vi "Acquisition.vi"(7 "CSM Name":string="CSM-Module") -> ()   [LabVIEW 2026, in "UI-压力.lvlib" / "Acquisition.lvlib"]
uses:
  Acquisition.lvlib
  Supports/Acquiring States.ctl
  Supports/Device Info.ctl
  Data ColndSave/Supports/Time and Data.ctl
  7c1bd55a-2ec8-456f-bad7-7e130b55c93f.vi
  d2ac0b8d-a34d-4c44-96e2-60a2cc9ef1dc.vi
  144ef8d5-f062-4612-a884-90947adc4c96.vi
  <userlib>/_NEVSTOP/Communicable State Machine(CSM)/AdvanceAPI/CSM - Revert Arguments-Safe String.vi
  <userlib>/_NEVSTOP/Communicable State Machine(CSM)/_Shared/Trim Single-line Text.vi
  <userlib>/_NEVSTOP/Communicable State Machine(CSM)/AdvanceAPI/CSM - Make String Arguments Safe.vi
  <userlib>/_NEVSTOP/Communicable State Machine(CSM)/AdvanceAPI/CSM - Break Down Multiple States String.vi
  <userlib>/_NEVSTOP/Communicable State Machine(CSM)/AdvanceAPI/CSM - Compact Multiple States.vi
  <userlib>/_NEVSTOP/Communicable State Machine(CSM)/AdvanceAPI/CSM - Keywords.vi
  <userlib>/_NEVSTOP/Communicable State Machine(CSM)/addons/API-String-Arugments-Support/_Support/Convert API String Arguments to Data(variant).vi
  <vilib>/Instr/_visa.llb/VISA Configure Serial Port (Instr).vi
  <userlib>/_NEVSTOP/Communicable State Machine(CSM)/addons/MassData-Parameter/_support/FGV-MassData(lvlibp).vi
  <userlib>/_NEVSTOP/Communicable State Machine(CSM)/Communicable State Machine.lvlib
  <userlib>/_NEVSTOP/Communicable State Machine(CSM)/addons/Loop-Support/CSM Loop Support.lvlib
  Data ColndSave/Data Collection and Save.lvlib
panel:
  out "Error Occurred":errorcluster
  out "State History":string
  in  "Exit":bool
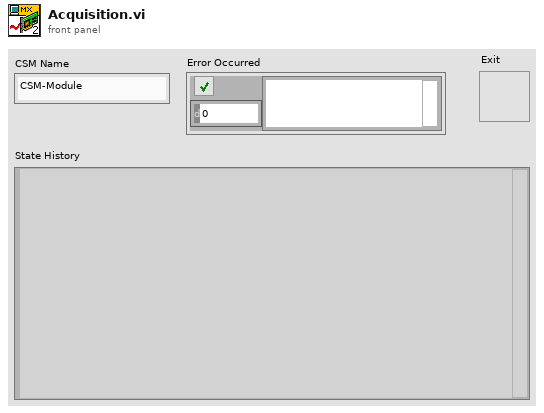
[diagram p1: front panel]
types:
  T1 = enum32{"Invalid", "Standard", "Closed", "Hidden", "Minimized", "Maximized"}
  T2 = enum32{"invalid app kind", "Development System", "Run Time System", "Student Edition", "Embedded LabVIEW", "Evaluation", "Custom"}
  T3 = typedef "UI-压力.lvlib/Acquisition.lvlib/Acquiring States.ctl" = enum16{"Idle", "Acquiring", "Error"}
  T4 = cluster{"波特率":u32, "数据位":u16, "校验":enum16{"None", "Odd", "Even", "Mark", "Space"}, "停止位":u16, "流控制":u16}
  T5 = typedef "Communicable State Machine.lvlib/_CSM_Response Source Message.ctl" = cluster{"‘State":string, "’Arguments":string, "’Error":errorcluster}
  T6 = cluster{"Current VI Reference":refnum<vi>, "Close Panel on Exit?":bool}
  T7 = typedef "UI-压力.lvlib/Device Info.ctl" = cluster{"USB Port":refnum<visa-resource-name>, "采集间隔(s)":dbl, "压力设备选择":bool}
  T8 = cluster{"Core":cluster{"Current VI Reference":refnum<vi>, "Close Panel on Exit?":bool}, "State":T3, "基本信息":T7, "采集时间":timestamp}
  T9 = typedef "Data Collection and Save.lvlib/Time and Data.ctl" = cluster{"采集时间":timestamp, "Data":dbl[]}
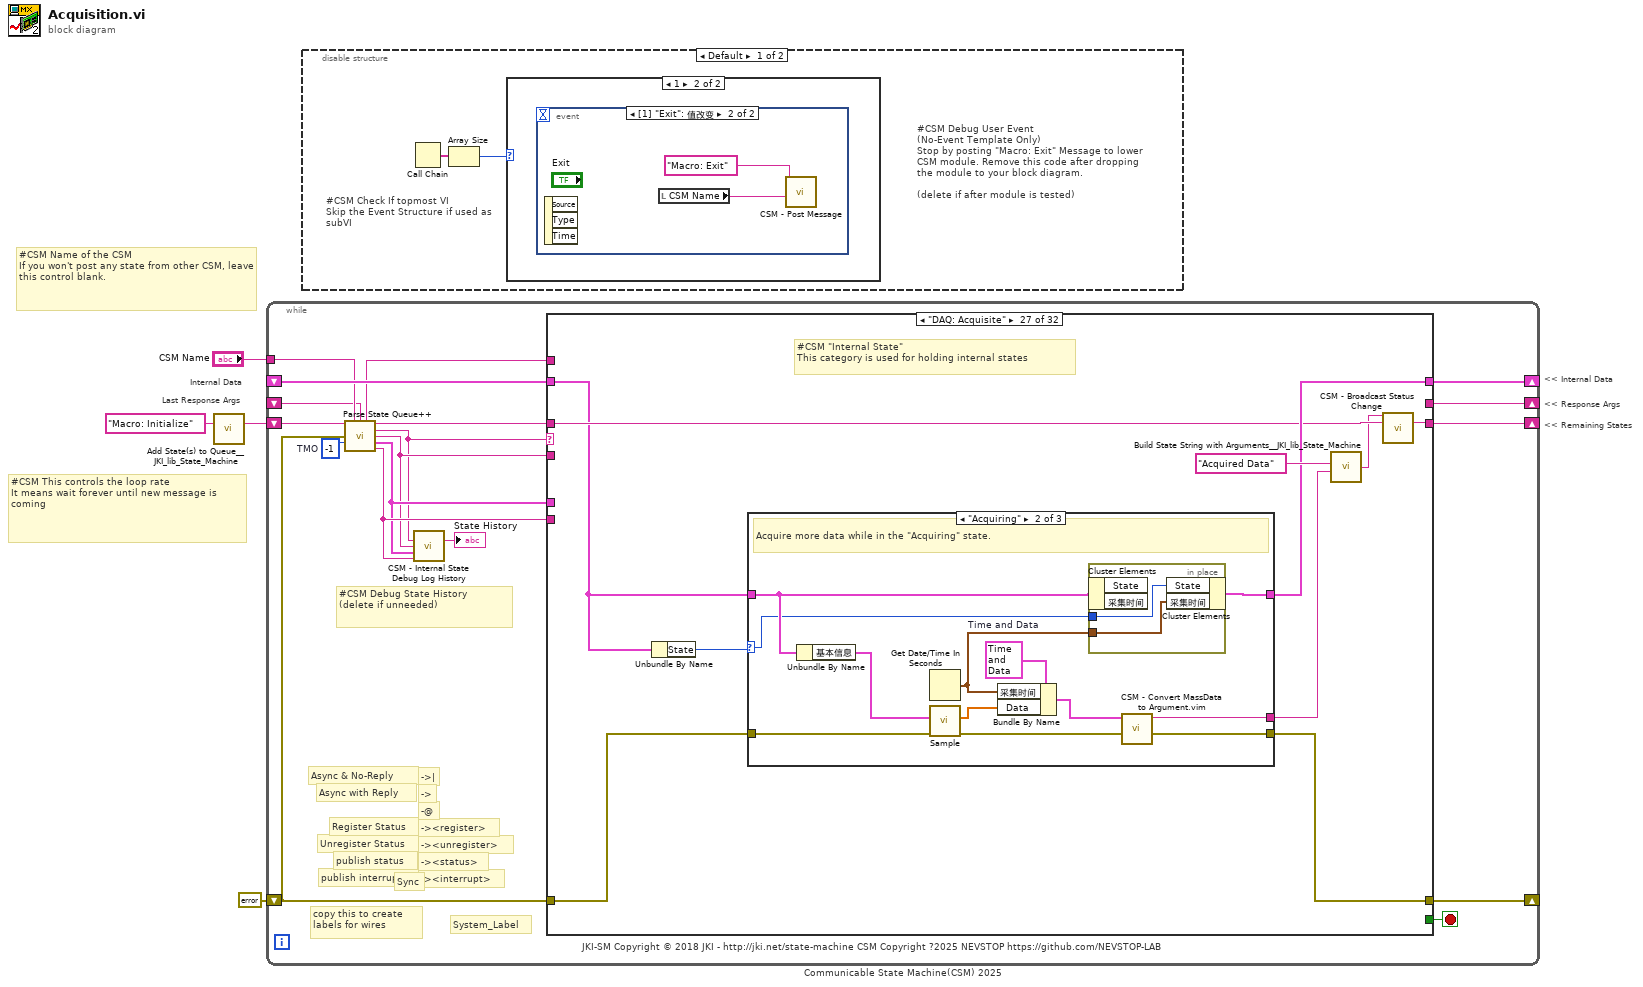
[diagram p0: block diagram]
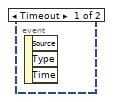
[diagram p3: hidden frame]
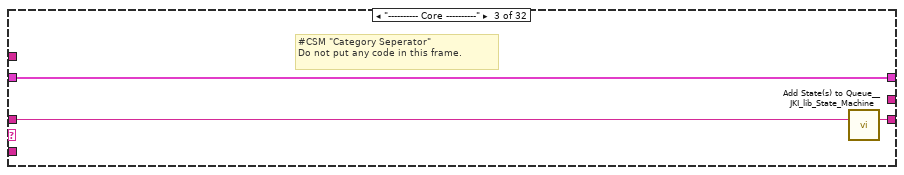
[diagram p7: hidden frame]
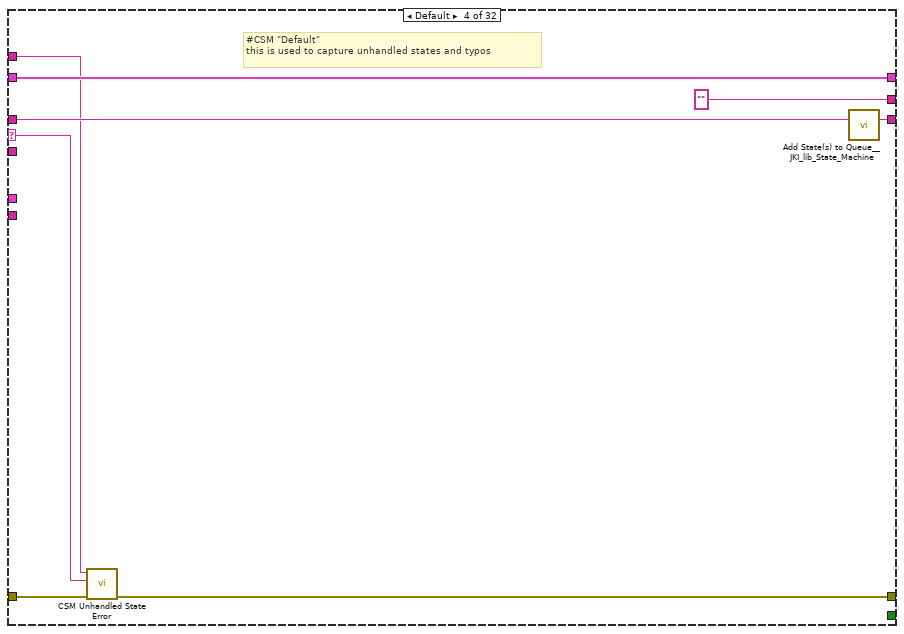
[diagram p8: hidden frame]
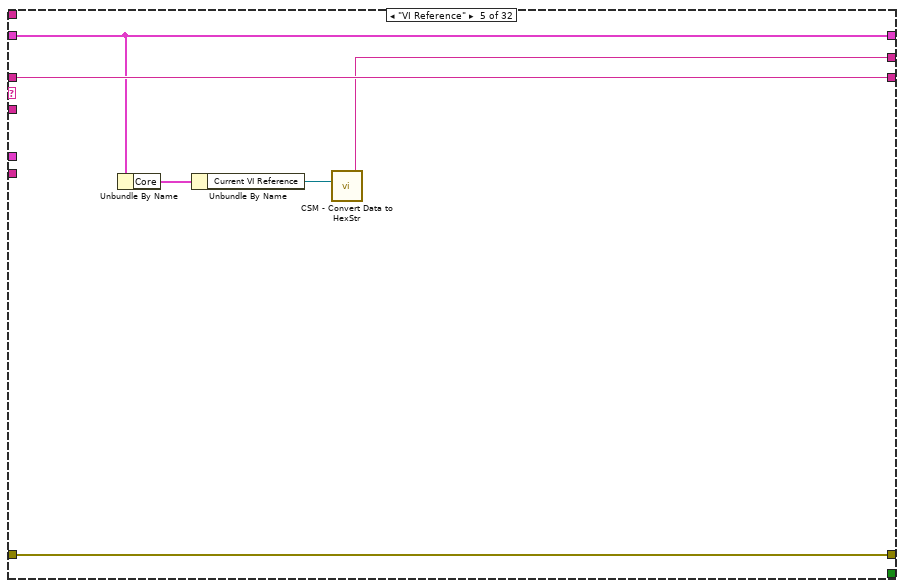
[diagram p9: hidden frame]
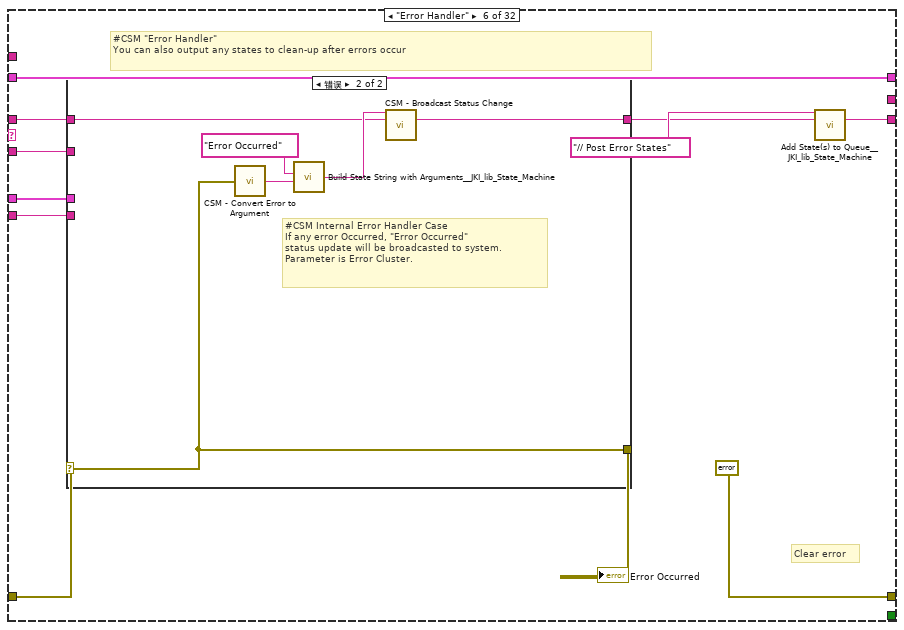
[diagram p10: hidden frame]
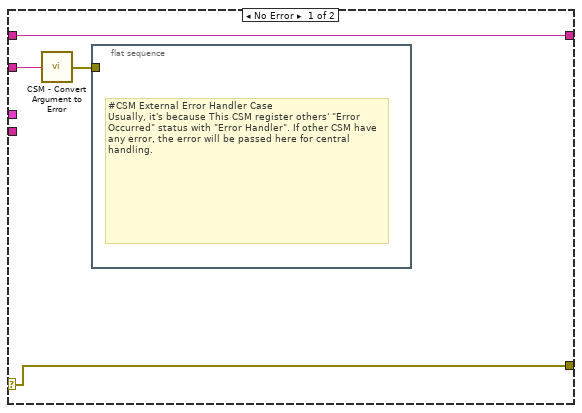
[diagram p11: hidden frame]
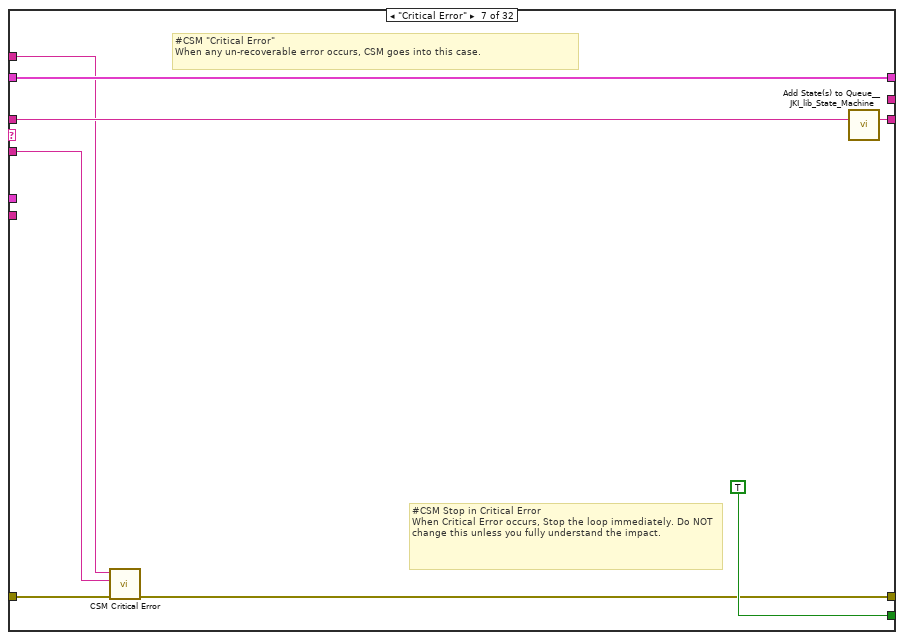
[diagram p12: hidden frame]
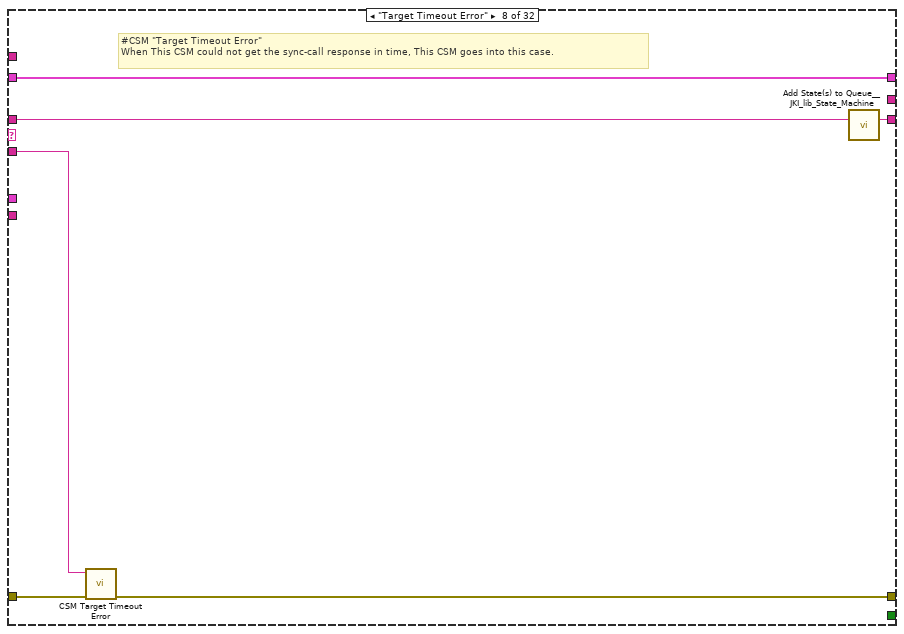
[diagram p13: hidden frame]
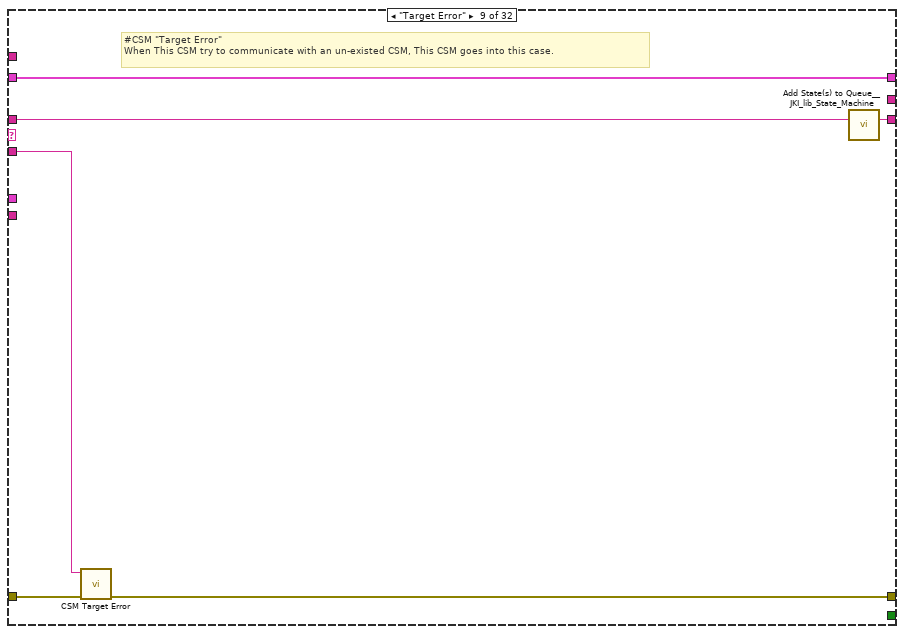
[diagram p14: hidden frame]
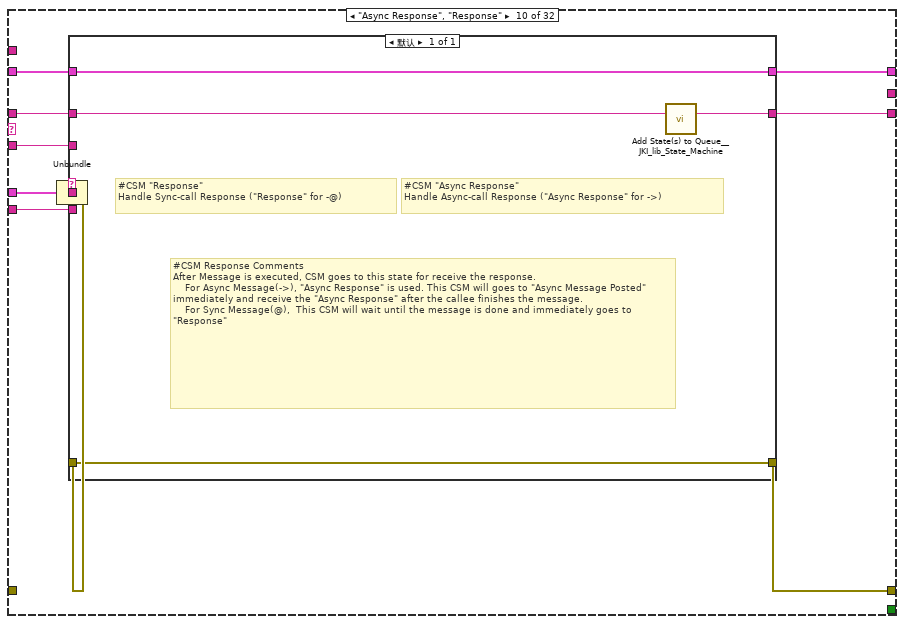
[diagram p15: hidden frame]
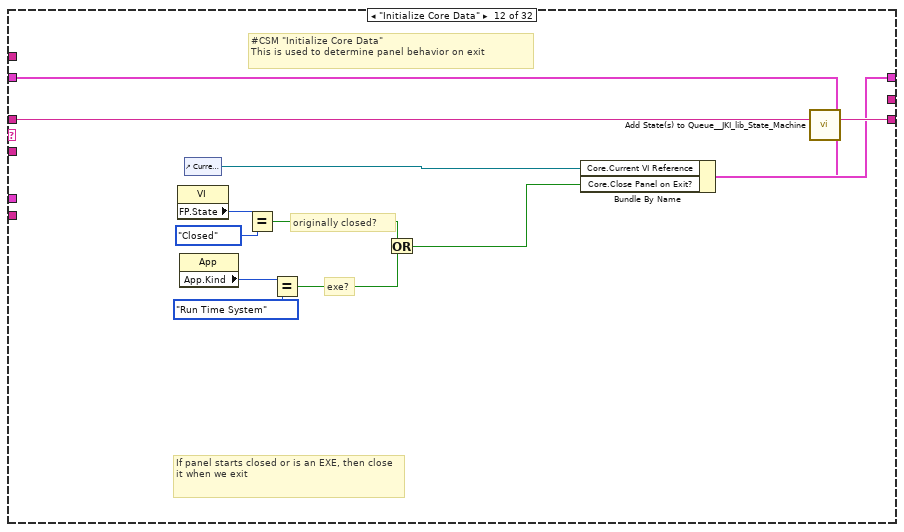
[diagram p17: hidden frame]
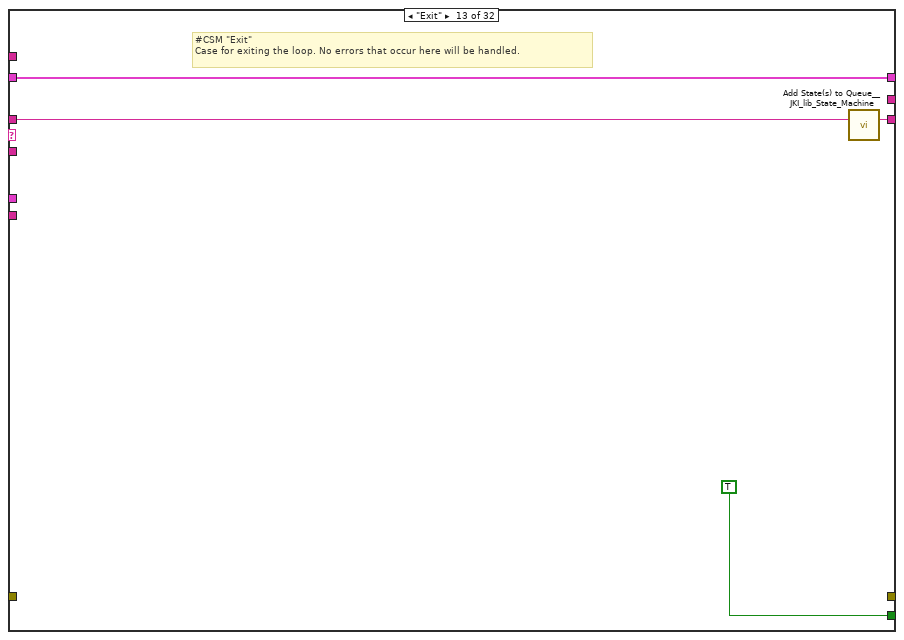
[diagram p18: hidden frame]
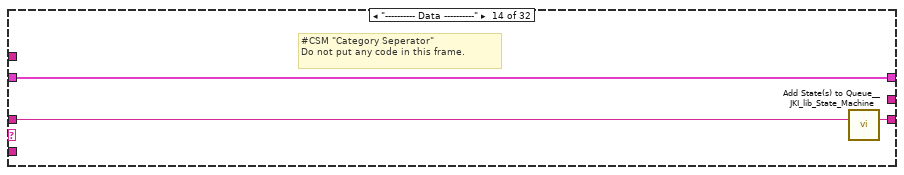
[diagram p19: hidden frame]
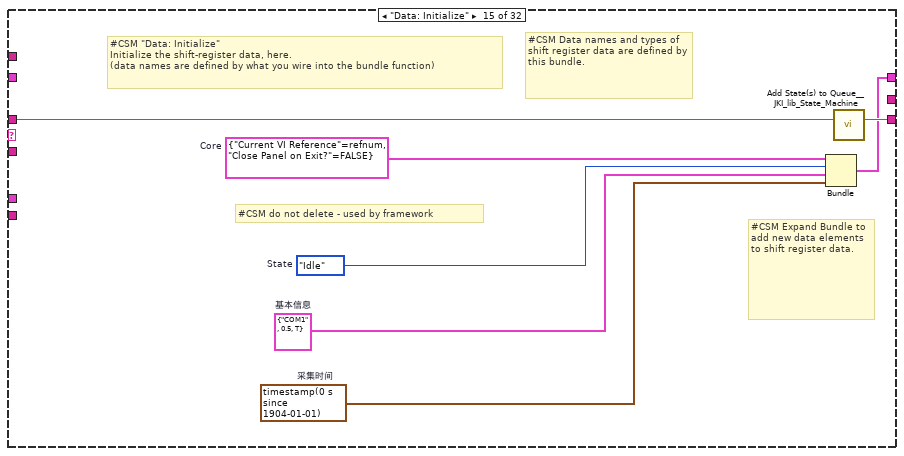
[diagram p20: hidden frame]
diagram:
  # "Last Response Args"
  # "Internal Data"
  # "#CSM Name of the CSM\nIf you won't post any state from other CSM, leave this control blank."
  # "#CSM This controls the loop rate\nIt means wait forever until new message is coming"
  # "<< Internal Data"
  # "<< Response Args"
  # "<< Remaining States"
  n1 = call <vilib>:"Add State(s) to Queue__JKI_lib_State_Machine.vi"("State(s) in (\"\")"="Macro: Initialize" ("Init State(\"Macro: Initialize\")")) -> ("States Out"=w1:string)  [unwired: 14 in]
  n2 = while "Communicable State Machine(CSM) 2025" {
    shift-right: [w17] -> _
    shift-left: _ -> [w16]
    shift-right: [w20] -> _
    shift-left: errorcluster {"status"=FALSE, "code"=0, "source"=""} ("error out") -> [w6]
    shift-right: [w19] -> _
    shift-left: w1 -> [w21]
    tunnel: "CSM Name" -> [w13]
    shift-right: [w14] -> _
    shift-left: _ -> [w8]
    stop <- w18 stop-if-true
    w15 = -1  # TMO
    # "#CSM Debug State History\n(delete if unneeded)"
    # "-><interrupt>"
    # "-><status>"
    # "-><unregister>"
    # "-><register>"
    # "-@"
    # "->"
    # "->|"
    # "publish interrupt"
    # "publish status"
    # "Unregister Status"
    # "Register Status"
    # "Sync"
    # "Async with Reply"
    # "Async & No-Reply"
    # "JKI-SM Copyright © 2018 JKI - http://jki.net/state-machine CSM Copyright ?2025 NEVSTOP https://github.com/NEVSTOP-LAB"
    # "copy this to create labels for wires"
    # "System_Label"
    n3 = call <userlib>:"Parse State Queue++.vi"("State Queue"=w21, "Name (\"\" to Use UUID)"=w13, "Response Arguments"=w8, "Previous Error"=w6, "Dequeue (1 ms)"=w15) -> ("Name Used"=w7:string, "Remaining States"=w22:string, "Current State"=w9:string, "Arguments"=w10:string, "Additional Information"=w11:T5, "Source CSM"=w12:string)  [unwired: 5 in]
    n4 = call <userlib>:"CSM - Internal State Debug Log History.vi"("State"=w9, "Arguments (\"\")"=w10, ">> Response Source Message >>"=w11, "Source (\"\")"=w12) -> ("Debug Log"=→"State History":string)  [unwired: 11 in]
    n5 = case shown="\"DAQ: Acquisite\"" w9 {
      selector: w9 -> [_ _ _ w33 _ _ _ _ _ _ _ _ _ _ _ _ _ _ _ _ _ _ _ _ _ _ _ _ _ _ w269 _]
      tunnel: w22 -> [w23 w26 w29 w37 w42 w48 w72 w78 w84 w94 w101 w113 w117 w120 w127 w130 w136 w139 w144 w153 w158 w163 w177 w182 w192 w205 w216 w247 w256 w258 w271 w274]
      tunnel: w10 -> [_ _ _ _ _ w47 w68 w75 w81 w88 _ _ _ _ _ _ _ _ _ _ _ w160 _ w186 _ _ _ _ _ _ w268 _]
      tunnel: w16 -> [w24 w25 w27 w35 w41 w53 w70 w76 w82 w92 w100 w107 w115 w118 _ w129 w131 w137 w142 w147 w157 w164 w179 w185 w190 w203 w213 w242 w253 w257 w260 w275]
      tunnel: [_ _ _ w30 w43 errorcluster {"status"=FALSE, "code"=0, "source"=""} ("error out") w65 w73 w79 w95 _ _ _ _ _ _ w132 _ w140 w145 _ w159 w175 w189 _ _ w218 _ _ w259 w272 w276] -> w20
      tunnel: w6 -> [_ _ _ w31 w43 w51 w66 w74 w80 _ _ _ _ _ _ _ w133 _ w140 w145 _ w159 w175 w189 _ _ w217 w241 _ w259 w272 w276]
      tunnel: [w23 w26 w28 w36 w42 w49 w71 w77 w83 w93 w101 w112 w116 w119 w126 w130 w135 w138 w143 w152 w158 w162 w178 w183 w191 w204 w214 w246 w255 w258 w270 w273] -> w19
      tunnel: [_ _ _ _ _ _ TRUE _ _ _ _ _ TRUE _ _ _ _ _ _ _ _ _ _ _ _ _ _ _ _ _ _ _] -> w18
      tunnel: [w24 w25 w27 w35 w41 w53 w70 w76 w82 w91 w100 w111 w115 w118 w125 w129 w131 w137 w142 w147 w157 w161 w179 w184 w190 w202 w219 w242 w252 w257 w260 w275] -> w17
      tunnel: w12 -> [_ _ _ _ _ w46 _ _ _ w89 _ _ _ _ _ _ _ _ _ _ _ _ _ _ _ _ _ _ _ _ _ _]
      tunnel: w11 -> [_ _ _ _ _ w45 _ _ _ w90 _ _ _ _ _ _ _ _ _ _ _ _ _ _ _ _ _ _ _ _ _ _]
      tunnel: [_ _ _ "" w38 _ _ _ _ _ _ _ _ _ _ _ _ _ _ _ _ _ _ _ _ _ _ _ _ _ _ _] -> w14
      tunnel: w7 -> [_ _ _ w32 _ _ w67 _ _ _ _ _ _ _ _ _ _ _ _ _ _ _ _ _ _ _ _ _ _ _ _ _]
      frame "", "Idle" {
        # "#CSM \"Idle/Event Handler\"\nexecutes when the state queue is empty"
      }
      frame "CSM Documentation" {
        # "#CSM State Syntax\n\n// Comment line, all text to the right of “//” will be ignored\n// Local Message Example\nDoSth: DoA >> Arguments\n\n// Sync Call Example\nAPI: xxxx >> Arguments -@ TargetModule\n\n// Async Call Example\nAPI: xxxx >> Arguments -> TargetModule\n\n// Async Call without Reply Example\nAPI: xxxx >> Arguments ->| TargetModule\n\n// Broadcast normal status:\nStatus >> StatusArguments  -><status>\n\n// Broadcast Interrupt status:\nInterrupt >> StatusArguments  -><interrupt>\n\n// Register Source Module's status to Handler Module\nStatus@Source Module >> Handler Module@Handler Module -><register>\n\n// Unegister Source Module's status\nStatus@Source Module >> Handler Module -><unregister>"
        # "#CSM README FIRST\n\nCommunicable State Machine(CSM) is a LabVIEW application framework that builds upon JKI State Machine(JKISM). It follows the pattern of JKISM and extends the keywords to describe message communication between modules, including concepts such as Sync-Message, Async-Message, Subscription/Unsubscription of status - essential elements for creating reusable code modules. For more information, please visit the CSM wiki: https://nevstop-lab.github.io/CSM-Wiki/\n\nFor instructions on JKI State Machine, visit: \n    http://jki.net/state-machine/\nFor information about CSM, visit: \n    https://github.com/NEVSTOP-LAB"
        # "#CSM \"Documentation\"\nCase for holding CSM Documenation"
      }
      frame "---------- Core ----------" {
        # "#CSM \"Category Seperator\"\nDo not put any code in this frame."
        n6 = call <vilib>:"Add State(s) to Queue__JKI_lib_State_Machine.vi"("State(s) in (\"\")"=w29) -> ("States Out"=w28:string)  [unwired: 14 in]
      }
      frame Default {
        # "#CSM \"Default\"\nthis is used to capture unhandled states and typos"
        n7 = call <userlib>:"CSM Unhandled State Error.vi"("error in (no error)"=w31, "Undefined State"=w33, "CSM Name"=w32) -> ("error out"=w30:errorcluster)  [unwired: 8 in]
        n8 = call <vilib>:"Add State(s) to Queue__JKI_lib_State_Machine.vi"("State(s) in (\"\")"=w37) -> ("States Out"=w36:string)  [unwired: 14 in]
      }
      frame "VI Reference" {
        n9 = Unbundle By Name(w41) -> ("Core"=w40:T6)
        n10 = Unbundle By Name(w40) -> ("Current VI Reference"=w39:refnum<vi>)
        n11 = call <userlib>:"CSM - Convert Data to HexStr.vi"("Variant"=w39) -> ("HEX String (0-9,A-F)"=w38:string)  [unwired: 8 in]
      }
      frame "Error Handler" {
        # "#CSM \"Error Handler\"\nYou can also output any states to clean-up after errors occur"
        # "Clear error"
        n12 = case shown="错误" w51 {
          selector: w51 -> [w55 w59]
          tunnel: [w58 w61] -> w50
          tunnel: w48 -> [w58 w60]
          tunnel: w47 -> [w57 _]
          tunnel: w46 -> [_ _]
          tunnel: w45 -> [_ _]
          tunnel: [w55 w59] -> w44
          frame No Error {
            n13 = call <userlib>:"CSM - Convert Argument to Error.vi"("Argument"=w57) -> ("Error"=w56:errorcluster)  [unwired: 4 in]
            n14 = flat-sequence {
              tunnel: w56 -> [_]
              frame #0 {
                # "#CSM External Error Handler Case\nUsually, it's because This CSM register others' \"Error Occurred\" status with \"Error Handler\". If other CSM have any error, the error will be passed here for central handling."
              }
            }
          }
          frame Error {
            # "#CSM Internal Error Handler Case \nIf any error Occurred, \"Error Occurred\" \nstatus update will be broadcasted to system.\nParameter is Error Cluster."
            n15 = call <userlib>:"CSM - Convert Error to Argument.vi"("Error"=w59) -> ("Argument"=w63:string)  [unwired: 4 in]
            n16 = call <vilib>:"Build State String with Arguments__JKI_lib_State_Machine.vi"("Arguments (\"\")"=w63, "State"="Error Occurred" ("Status with Arguments")) -> ("State with Arguments"=w62:string)  [unwired: 4 in]
            n17 = call <userlib>:"CSM - Broadcast Status Change.vi"("Status With Arguments"=w62, "State Queue"=w60) -> ("Remaining States"=w61:string)  [unwired: 13 in]
          }
        }
        "Error Occurred" <- w44
        n18 = call <vilib>:"Add State(s) to Queue__JKI_lib_State_Machine.vi"("State(s) in Front (\"\")"="// Post Error States", "State(s) in (\"\")"=w50) -> ("States Out"=w49:string)  [unwired: 13 in]
      }
      frame "Critical Error" {
        # "#CSM \"Critical Error\"\nWhen any un-recoverable error occurs, CSM goes into this case."
        # "#CSM Stop in Critical Error\nWhen Critical Error occurs, Stop the loop immediately. Do NOT change this unless you fully understand the impact."
        n19 = call <userlib>:"CSM Critical Error.vi"("error in (no error)"=w66, "Arugments (As Reason)"=w68, "CSM Name"=w67) -> ("error out"=w65:errorcluster)  [unwired: 8 in]
        n20 = call <vilib>:"Add State(s) to Queue__JKI_lib_State_Machine.vi"("State(s) in (\"\")"=w72) -> ("States Out"=w71:string)  [unwired: 14 in]
      }
      frame "Target Timeout Error" {
        # "#CSM \"Target Timeout Error\"\nWhen This CSM could not get the sync-call response in time, This CSM goes into this case."
        n21 = call <userlib>:"CSM Target Timeout Error.vi"("error in (no error)"=w74, "Arguments (As CSM Name)"=w75) -> ("error out"=w73:errorcluster)  [unwired: 9 in]
        n22 = call <vilib>:"Add State(s) to Queue__JKI_lib_State_Machine.vi"("State(s) in (\"\")"=w78) -> ("States Out"=w77:string)  [unwired: 14 in]
      }
      frame "Target Error" {
        # "#CSM \"Target Error\"\nWhen This CSM try to communicate with an un-existed CSM, This CSM goes into this case."
        n23 = call <userlib>:"CSM Target Error.vi"("error in (no error)"=w80, "Arguments (As CSM Name)"=w81) -> ("error out"=w79:errorcluster)  [unwired: 9 in]
        n24 = call <vilib>:"Add State(s) to Queue__JKI_lib_State_Machine.vi"("State(s) in (\"\")"=w84) -> ("States Out"=w83:string)  [unwired: 14 in]
      }
      frame "Async Response", "Response" {
        n25 = Unbundle(w90) -> ("‘State"=w87:string, "’Arguments"=w86:string, "’Error"=w85:errorcluster)
        n26 = case shown="默认" w87 {
          tunnel: [w96] -> w93
          tunnel: w94 -> [w97]
          tunnel: [w99] -> w91
          tunnel: w92 -> [w99]
          tunnel: [w98] -> w95
          tunnel: w85 -> [w98]
          tunnel: w89 -> [_]
          tunnel: w88 -> [_]
          tunnel: w86 -> [_]
          frame 默认 {
            # "#CSM \"Async Response\"\nHandle Async-call Response (\"Async Response\" for ->)"
            # "#CSM \"Response\"\nHandle Sync-call Response (\"Response\" for -@)"
            # "#CSM Response Comments\nAfter Message is executed, CSM goes to this state for receive the response.\n    For Async Message(->), \"Async Response\" is used. This CSM will goes to \"Async Message Posted\" immediately and receive the \"Async Response\" after the callee finishes the message.\n    For Sync Message(@),  This CSM will wait until the message is done and immediately goes to \"Response\""
            n27 = call <vilib>:"Add State(s) to Queue__JKI_lib_State_Machine.vi"("State(s) in (\"\")"=w97) -> ("States Out"=w96:string)  [unwired: 14 in]
          }
        }
      }
      frame "Async Message Posted" {
        # "#CSM \"Async Message Posted\"\nAfter Async Message is posted (-> or ->| ), CSM goes to this state for post-action.\nYou can use Argument - State to tell which Async Message is called."
      }
      frame "Initialize Core Data" {
        # "#CSM \"Initialize Core Data\"\nThis is used to determine panel behavior on exit"
        # "originally closed?"
        # "exe?"
        # "If panel starts closed or is an EXE, then close it when we exit"
        n28 = property class="VI"() -> ("FP.State"=w104:T1)  [unwired: 2 in, 2 out]
        n29 = property class="App"() -> ("App.Kind"=w110:T2)  [unwired: 2 in, 2 out]
        n30 = control-ref of="Current VI Reference"() -> (w105:refnum<vi>)
        n31 = Equal?(x=w104, y=T1."Closed" ("Front Panel Window:State")) -> (x = y?=w102:bool)
        n32 = Equal?(x=w110, y=T2."Run Time System" ("Application:Kind")) -> (x = y?=w108:bool)
        n33 = Or(x=w102, y=w108) -> (x .or. y?=w106:bool)
        n34 = Bundle By Name(cluster=w107, "Core.Current VI Reference"=w105, "Core.Close Panel on Exit?"=w106) -> (w111:T8)
        n35 = call <vilib>:"Add State(s) to Queue__JKI_lib_State_Machine.vi"("State(s) in (\"\")"=w113) -> ("States Out"=w112:string)  [unwired: 14 in]
      }
      frame "Exit" {
        # "#CSM \"Exit\"\nCase for exiting the loop. No errors that occur here will be handled."
        n36 = call <vilib>:"Add State(s) to Queue__JKI_lib_State_Machine.vi"("State(s) in (\"\")"=w117) -> ("States Out"=w116:string)  [unwired: 14 in]
      }
      frame "---------- Data ----------" {
        # "#CSM \"Category Seperator\"\nDo not put any code in this frame."
        n37 = call <vilib>:"Add State(s) to Queue__JKI_lib_State_Machine.vi"("State(s) in (\"\")"=w120) -> ("States Out"=w119:string)  [unwired: 14 in]
      }
      frame "Data: Initialize" {
        w121 = T7 {"USB Port"="COM1", "采集间隔(s)"=0.5, "压力设备选择"=TRUE}  # 基本信息
        w122 = timestamp(0 s since 1904-01-01)  # 采集时间
        w123 = Acquiring_States."Idle"  # State
        w124 = T6 {"Current VI Reference"=refnum, "Close Panel on Exit?"=FALSE}  # Core
        # "#CSM \"Data: Initialize\"\nInitialize the shift-register data, here.\n(data names are defined by what you wire into the bundle function)"
        # "#CSM do not delete - used by framework"
        # "#CSM Expand Bundle to add new data elements to shift register data."
        # "#CSM Data names and types of shift register data are defined by this bundle."
        n38 = Bundle("Core"=w124, "State"=w123, "基本信息"=w121, "采集时间"=w122) -> (w125:T8)  [unwired: 1 in]
        n39 = call <vilib>:"Add State(s) to Queue__JKI_lib_State_Machine.vi"("State(s) in (\"\")"=w127) -> ("States Out"=w126:string)  [unwired: 14 in]
      }
      frame "Data: Update Indicators" {
        n40 = local write "Error Occurred"(errorcluster {"status"=FALSE, "code"=0, "source"=""} ("错误常量")) -> ()
      }
      frame "Data: Cleanup" {
        # "#CSM \"Data: Cleanup\"\nCleanup any data and references, here.\n(this is called automatically, by the Macro: Exit)"
        n41 = Unbundle By Name(w131) -> ("Core.Current VI Reference"=w134:refnum<vi>)
        n42 = Close Reference(reference=w134, error in (no error)=w133) -> (error out=w132:errorcluster)
        n43 = call <vilib>:"Add State(s) to Queue__JKI_lib_State_Machine.vi"("State(s) in (\"\")"=w136) -> ("States Out"=w135:string)  [unwired: 14 in]
      }
      frame "---------- Macro ----------" {
        # "#CSM \"Category Seperator\"\nDo not put any code in this frame."
        n44 = call <vilib>:"Add State(s) to Queue__JKI_lib_State_Machine.vi"("State(s) in (\"\")"=w139) -> ("States Out"=w138:string)  [unwired: 14 in]
      }
      frame "Macro: Initialize" {
        # "#CSM \"Macro: Initialize\"\nInitialization Macro (This is called once, when the VI starts)"
        n45 = call <vilib>:"Add State(s) to Queue__JKI_lib_State_Machine.vi"("State(s) in Front (\"\")"="Data: Initialize\nInitialize Core Data\nData: Update Indicators", "State(s) in (\"\")"=w144) -> ("States Out"=w143:string)  [unwired: 13 in]
      }
      frame "Macro: Exit" {
        # "#CSM \"Macro: Exit\"\nExit Macro (This is called once, when the VI exits)"
        n46 = Unbundle By Name(w147) -> ("State"=w148:T3)
        n47 = case shown="\"Acquiring\"" w148 {
          tunnel: ["" "Break Continuous" ""] -> w146
          frame "Idle", Default {
          }
          frame "Acquiring" {
          }
          frame "Error" {
          }
        }
        n48 = call <vilib>:"Add State(s) to Queue__JKI_lib_State_Machine.vi"("State(s) in Front (\"\")"="//Exit Sub-Modules ", "State(s) in (\"\")"=w146, "State(s) at Back (\"\")"="Data: Cleanup\nExit") -> ("States Out"=w150:string)  [unwired: 12 in]
        n49 = call <vilib>:"Add State(s) to Queue__JKI_lib_State_Machine.vi"("State(s) in Front (\"\")"=w150, "State(s) in (\"\")"=w153) -> ("States Out"=w152:string)  [unwired: 13 in]
      }
      frame "---------- API ----------" {
        # "#CSM \"Category Seperator\"\nDo not put any code in this frame."
      }
      frame "API: Start" {
        # "#CSM API Example\nCopy/Rename this case for your own API"
        # "#CSM API Example\nCopy/Rename this case for your own API"
        n50 = Unbundle By Name(w164) -> ("State"=w167:T3)
        n51 = Unbundle By Name(w164) -> ("基本信息"=w170:T7)
        n52 = case shown="\"Idle\"" w167 {
          selector: w167 -> [_ w173 w174]
          tunnel: [Acquiring_States."Acquiring" ("Acquisition State") w173 w174] -> w166
          tunnel: ["DAQ: Initialize \nDAQ: Acquisite\nContinuous Check >> DAQ: Acquisite -><loop> \nDAQ: Close " ("State(s) in Front (\"\")") _ _] -> w168
          frame "Idle" {
            # "If the system is idle, start the acquisition."
          }
          frame "Acquiring" {
            # "The system is already acquiring. Ignore the \"Start\" message."
          }
          frame "Error" {
          }
        }
        n53 = local write "Error Occurred"(errorcluster {"status"=FALSE, "code"=0, "source"=""} ("错误常量")) -> ()
        n54 = call "Convert API String Arguments to Data.vim"("Reference Type"=w170, "API String"=w160) -> ("Data"=w169:T7)  [unwired: 6 in, 1 out]
        n55 = call <userlib>:"CSMLS - Define Loop State(s).vi"("Loop States"=w168, "States Queue"=w163) -> ("Remaining States"=w162:string)  [unwired: 13 in]
        n56 = Bundle By Name(cluster=w164, "State"=w166, "基本信息"=w169) -> (w161:T8)
      }
      frame "API: Stop" {
        # "#CSM API Example\nCopy/Rename this case for your own API"
        n57 = Unbundle By Name(w179) -> ("State"=w180:T3)
        n58 = case shown="\"Acquiring\"" w180 {
          tunnel: [_ "Break Continuous" ("State(s) in Front (\"\")") _] -> w176
          frame "Idle" {
            # "The system is already idle. Ignore the \"Stop\" message."
          }
          frame "Acquiring" {
            # "If the system is acquiring, stop the acquisition."
          }
          frame "Error" {
          }
        }
        n59 = call <vilib>:"Add State(s) to Queue__jki_lib_state_machine.vi"("State(s) in Front (\"\")"=w176, "State(s) in (\"\")"=w177) -> ("States Out"=w178:string)  [unwired: 13 in]
      }
      frame "API: Sample Interval" {
        n60 = call "Convert API String Arguments to Data.vim"("Reference Type"=0.0, "API String"=w186) -> ("Data"=w187:dbl)  [unwired: 6 in, 1 out]
        n61 = Bundle By Name(cluster=w185, "基本信息.采集间隔(s)"=w187) -> (w184:T8)
        n62 = call <vilib>:"Add State(s) to Queue__jki_lib_state_machine.vi"("State(s) in (\"\")"=w182) -> ("States Out"=w183:string)  [unwired: 14 in]
      }
      frame "---------- DAQ ----------" {
        # "#CSM \"Category Seperator\"\nDo not put any code in this frame."
        n63 = call <vilib>:"Add State(s) to Queue__JKI_lib_State_Machine.vi"("State(s) in (\"\")"=w192) -> ("States Out"=w191:string)  [unwired: 14 in]
      }
      frame "DAQ: Initialize" {
        # "#CSM \"Category Seperator\"\nDo not put any code in this frame."
        n64 = Unbundle By Name(w203) -> ("基本信息.压力设备选择"=w195:bool, "基本信息.USB Port"=w194:refnum<visa-resource-name>)
        n65 = Unbundle By Name(T4 {"波特率"=9600, "数据位"=8, "校验"=enum."None", "停止位"=10, "流控制"=0} ("串口设置")) -> ("波特率"=w201:u32, "数据位"=w200:u16, "校验"=w199:enum16{"None", "Odd", "Even", "Mark", "Space"}, "停止位"=w198:u16, "流控制"=w197:u16)
        n66 = case shown="True" w195 {
          tunnel: w194 -> [_ w207]
          frame False {
          }
          frame True {
            n67 = flat-sequence {
              tunnel: w207 -> [w208]
              tunnel: [w208] -> w206
              tunnel: w206 -> [w210]
              frame #0 {
                n68 = call "AO 薄膜(子VI) - PS2.vi"("电压"=5.0 ("Double"), "VISA资源名称"=w208) -> ()  [unwired: 9 in, 1 out]
              }
              frame #1 {
                n69 = call "AO 薄膜(子VI) - PS2.vi"("电压"=5.0 ("Double"), "VISA资源名称"=w210) -> ()  [unwired: 9 in, 1 out]
                n70 = Wait (ms)(milliseconds to wait=u32 300 ("等待时间（毫秒）")) -> ()  [unwired: 1 out]
              }
            }
          }
        }
        n71 = call-poly "VISA Configure Serial Port"("VISA resource name"=w194, "baud rate (9600)"=w201, "data bits (8)"=w200, "parity (0:none)"=w199, "stop bits (10: 1 bit)"=w198, "flow control (0:none)"=w197) -> ("VISA resource name out"=w193:refnum<visa-resource-name>)  [unwired: 3 in, 6 out]
        n72 = Bundle By Name(cluster=w203, "基本信息.USB Port"=w193) -> (w202:T8)
        n73 = call <vilib>:"Add State(s) to Queue__JKI_lib_State_Machine.vi"("State(s) in (\"\")"=w205) -> ("States Out"=w204:string)  [unwired: 14 in]
      }
      frame "DAQ: Acquisite" {
        # "#CSM \"Internal State\"\nThis category is used for holding internal states"
        n74 = Unbundle By Name(w213) -> ("State"=w222:T3)
        n75 = case shown="\"Acquiring\"" w222 {
          selector: w222 -> [_ w226 _]
          tunnel: [w224 w235 w240] -> w218
          tunnel: w217 -> [w224 w234 w240]
          tunnel: [w223 w227 w239] -> w219
          tunnel: w213 -> [w223 w228 w239]
          tunnel: [_ w236 _] -> w220
          frame "Idle" {
            # "Ignore \"Acquire\" messages when the acquisition is idle."
          }
          frame "Acquiring" {
            w232 = T9 {"采集时间"=timestamp(0 s since 1904-01-01), "Data"=[]}  # Time and Data
            # "Acquire more data while in the \"Acquiring\" state."
            n76 = Unbundle By Name(w228) -> ("基本信息"=w229:T7)
            n77 = Get Date/Time In Seconds() -> (seconds since 1Jan1904=w225:timestamp)
            n78 = call "Sample.vi"("Error In"=w234, "基本信息"=w229) -> ("Error Out"=w233:errorcluster, "Data"=w230:dbl[])  [unwired: 8 in]
            n79 = Bundle By Name(cluster=w232, "采集时间"=w225, "Data"=w230) -> (w231:T9)
            n80 = in-place {
              in-place-border: w226 -> [w238]
              in-place-border: w225 -> [w237]
              n81 = in-place-cluster #1(w228) -> ()  [unwired: 2 out]
              n82 = in-place-cluster #1("State"=w238, "采集时间"=w237) -> (w227:T8)
            }
            n83 = call "CSM - Convert MassData to Argument.vim"("error in (no error)"=w233, "Data"=w231) -> ("error out"=w235:errorcluster, "MassData Argument"=w236:string)  [unwired: 6 in]
          }
          frame "Error" {
          }
        }
        n84 = call <vilib>:"Build State String with Arguments__JKI_lib_State_Machine.vi"("Arguments (\"\")"=w220, "State"="Acquired Data" ("Status with Arguments")) -> ("State with Arguments"=w215:string)  [unwired: 4 in]
        n85 = call <userlib>:"CSM - Broadcast Status Change.vi"("Status With Arguments"=w215, "State Queue"=w216) -> ("Remaining States"=w214:string)  [unwired: 13 in]
      }
      frame "DAQ: Stop" {
        # "#CSM \"Internal State\"\nThis category is used for holding internal states"
        n86 = Unbundle By Name(w242) -> ("基本信息.压力设备选择"=w245:bool, "基本信息.USB Port"=w244:refnum<visa-resource-name>)
        n87 = case shown="True" w245 {
          tunnel: w241 -> [w248 w250]
          tunnel: [w248 w250] -> w243
          tunnel: w244 -> [_ w249]
          frame False {
          }
          frame True {
            n88 = call "AO 薄膜(子VI) - PS2.vi"("电压"=0.0 ("Double"), "VISA资源名称"=w249) -> ()  [unwired: 9 in, 1 out]
          }
        }
        n89 = VISA Close(VISA resource name=w244, error in (no error)=w243) -> ()  [unwired: 1 out]
        n90 = call <vilib>:"Add State(s) to Queue__JKI_lib_State_Machine.vi"("State(s) in (\"\")"=w247) -> ("States Out"=w246:string)  [unwired: 14 in]
      }
      frame "DAQ: Close" {
        w254 = Acquiring_States."Idle"  # State
        # "#CSM \"Internal State\"\nThis category is used for holding internal states"
        n91 = Bundle By Name(cluster=w253, "State"=w254) -> (w252:T8)
        n92 = call <vilib>:"Add State(s) to Queue__JKI_lib_State_Machine.vi"("State(s) in (\"\")"=w256) -> ("States Out"=w255:string)  [unwired: 14 in]
      }
      frame "---------- Loop ----------" {
      }
      frame "Continuous Check" {
        n93 = Unbundle By Name(w260) -> ("基本信息.采集间隔(s)"=w267:dbl, "采集时间"=w264:timestamp)
        n94 = Get Date/Time In Seconds() -> (seconds since 1Jan1904=w265:timestamp)
        n95 = Multiply(x=u32 1000 ("y"), y=w267) -> (x*y=w263:dbl)
        n96 = Subtract(x=w265, y=w264) -> (x-y=w262:dbl)
        n97 = Subtract(x=w263, y=w262) -> (x-y=w261:dbl)
        n98 = Wait (ms)(milliseconds to wait=w261) -> ()  [unwired: 1 out]
        n99 = call <userlib>:"CSMLS - Append Continuous State.vi"("Loop State(s) And Arguments"=w268, "Continous Arguments (\"\")"=w268, "Continous State"=w269, "States Queue"=w271) -> ("Remaining States"=w270:string)  [unwired: 7 in]
      }
      frame "Break Continuous" {
        n100 = call <userlib>:"CSMLS - Remove Loop Tag to Break.vi"("States Queue"=w274) -> ("Remaining States"=w273:string)  [unwired: 10 in]
      }
    }
  }
  n101 = disable-structure shown="Default" {
    frame condition #0 (active) {
      # "#CSM Check If topmost VI\nSkip the Event Structure if used as subVI"
      # "#CSM Debug User Event\n(No-Event Template Only)\nStop by posting \"Macro: Exit\" Message to lower CSM module. Remove this code after dropping the module to your block diagram. \n\n(delete if after module is tested)"
      n102 = Call Chain() -> (call chain=w278:string[])
      n103 = Array Size(array=w278) -> (size(s)=w277:i32)
      n104 = case shown="1" w277 {
        frame Default {
        }
        frame 1 {
          n105 = event shown="[1] \"Exit\": 值改变" {
            selector: _ -> [_ _]
            dyn-events: _ -> [_ _]
            timeout: _ -> [_ _]
            event Timeout {
              n106 = event-data() -> ()  [unwired: 1 in, 3 out]
            }
            event "Exit": Value Change {
              n107 = event-data() -> ()  [unwired: 1 in, 3 out]
              n108 = local read "CSM Name"() -> (w280:string)
              n109 = call <userlib>:"CSM - Post Message.vi"("Target Module"=w280, "State"="Macro: Exit" ("States")) -> ()  [unwired: 9 in, 1 out]
            }
          }
        }
      }
    }
    frame condition #1 {
    }
  }
